vi "Remove common path.vi"(11 "VI Paths In":path[](array[path])) -> (3 "VI Paths Out":path[](array[path]))   [LabVIEW 2019, in "Language Selection.lvlib"]
doc: "Removes the common leading folder from all paths, so that only the differing parts remain.\n- - -\nCopyright (c) 2026, Merecs Engineering GmbH"
uses:
  Language Selection.lvlib
panel:
  # "Connector Pane"
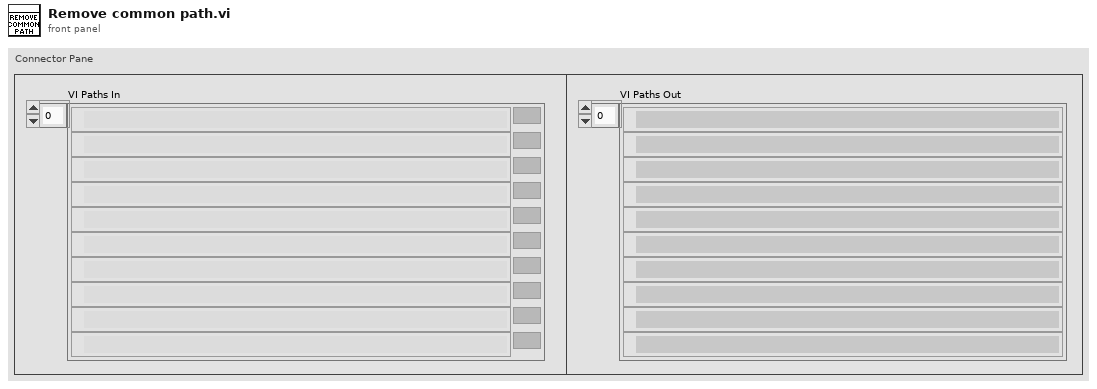
[diagram p1: front panel]
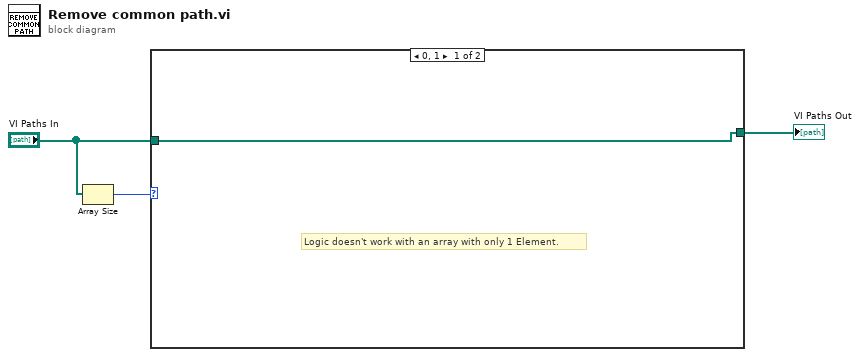
[diagram p0: block diagram]
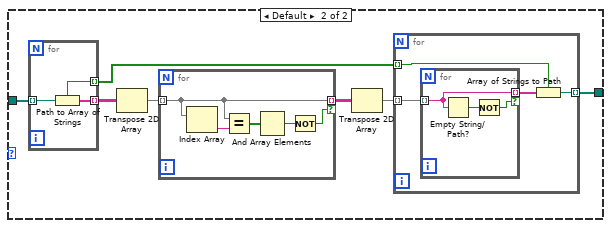
[diagram p2: hidden frame]
diagram:
  n1 = Array Size(array="VI Paths In") -> (size(s)=w1:i32)
  n2 = case shown="0, 1" w1 {
    tunnel: [w4 w10] -> w3
    tunnel: "VI Paths In" -> [w4 w5]
    frame 0, 1 {
      # "Logic doesn't work with an array with only 1 Element."
    }
    frame Default {
      n3 = for {
        tunnel: w5 -> [w26] mode=indexing
        tunnel: [w25] -> w6 mode=indexing
        tunnel: [w24] -> w11 mode=indexing
        n4 = Path to Array of Strings(0:w26) -> (1:w24:bool, 2:w25:string[])
      }
      n5 = Transpose 2D Array(2D array=w6) -> (transposed array=w7:string[][])
      n6 = for {
        tunnel: w7 -> [w22] mode=indexing
        tunnel: [w22] -> w8 mode=indexing if=w19
        n7 = Index Array(array=w22) -> (element=w23:string)  [unwired: 1 in]
        n8 = Equal?(x=w22, y=w23) -> (x = y?=w21:bool[])
        n9 = And Array Elements(Boolean array=w21) -> (logical AND=w20:bool)
        n10 = Not(x=w20) -> (.not. x?=w19:bool)
      }
      n11 = Transpose 2D Array(2D array=w8) -> (transposed array=w9:string[][])
      n12 = for {
        tunnel: w9 -> [w13] mode=indexing
        tunnel: [w15] -> w10 mode=indexing
        tunnel: w11 -> [w14] mode=indexing
        n13 = for {
          tunnel: w13 -> [w18] mode=indexing
          tunnel: [w18] -> w12 mode=indexing if=w16
          n14 = Empty String/Path?(string/path=w18) -> (empty?=w17:bool)
          n15 = Not(x=w17) -> (.not. x?=w16:bool)
        }
        n16 = Array of Strings to Path(0:w12, 1:w14) -> (2:w15:path)
      }
    }
  }
  "VI Paths Out" <- w3
